vi "C_CAN_Serialize.vi"(6 "brs":bool, 7 "ide":bool, 8 "error in (no error)":errorcluster, 9 "fdf":bool, 10 "id":u32 format="%.0x", 11 "data":u8[](array[numeric]) format="%.0x") -> (0 "error out":errorcluster, 3 "payload":u8[](array[numeric]) format="%.0x")   [LabVIEW 2021, in "CANsub_C.lvlib"]
doc: "Serializes one CAN or CAN FD frame into the CANsub transmit payload (header + data). Classic: at most 8 data bytes. FD: at most 64, zero-padded to the next FD length. Standard IDs are masked to 11 bits."
uses:
  CANsub_C.lvlib
  codec_vis/CANsub_Codec.lvlib
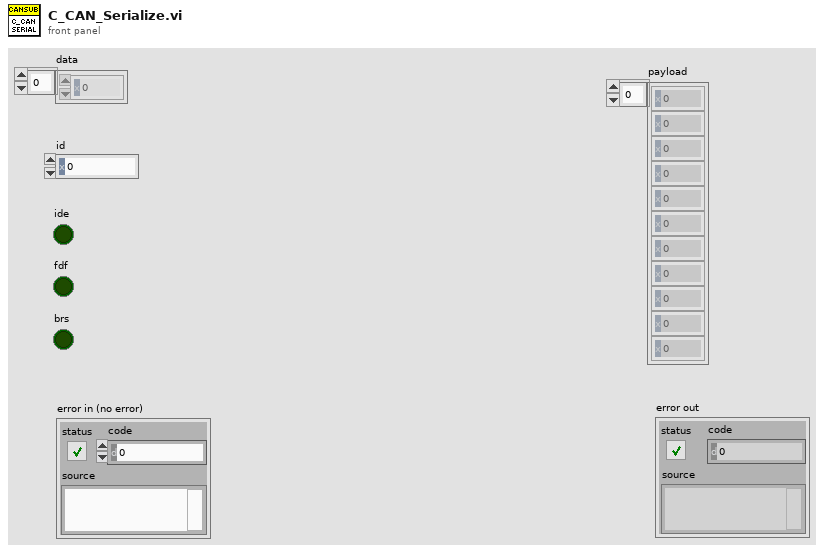
[diagram p1: front panel]
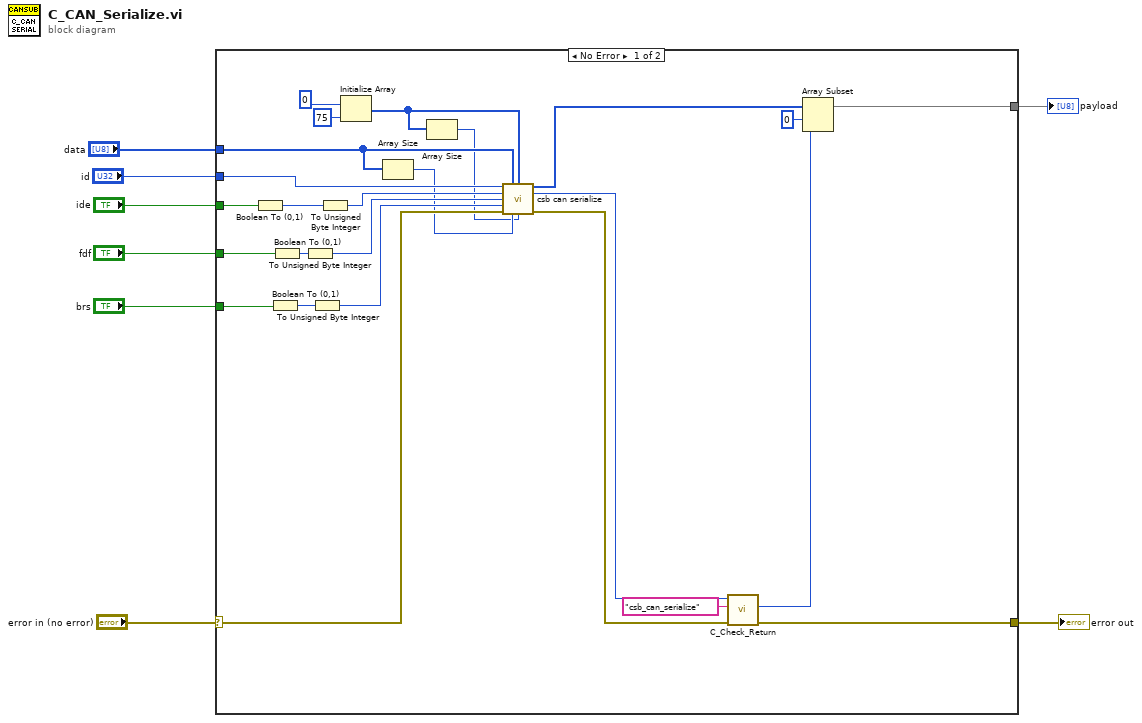
[diagram p0: block diagram]
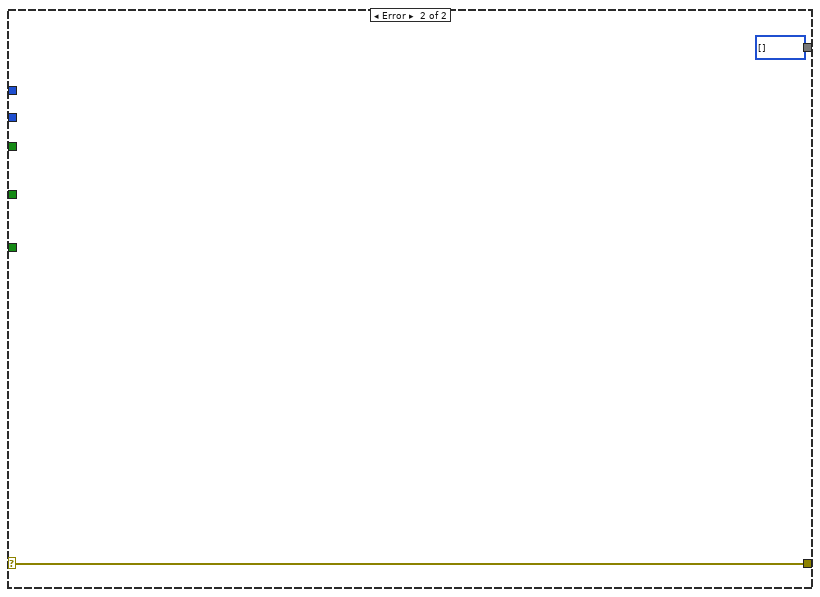
[diagram p2: hidden frame]
diagram:
  n1 = case shown="No Error" "error in (no error)" {
    selector: "error in (no error)" -> [w31 w35]
    tunnel: [w29 w35] -> w7
    tunnel: [w11 u8[] [] ("payload")] -> w6
    tunnel: "ide" -> [w26 _]
    tunnel: "fdf" -> [w25 _]
    tunnel: "brs" -> [w24 _]
    tunnel: "id" -> [w17 _]
    tunnel: "data" -> [w15 _]
    frame No Error {
      n2 = Boolean To (0,1)(Boolean=w26) -> (0, 1=w21:i16)
      n3 = Boolean To (0,1)(Boolean=w24) -> (0, 1=w23:i16)
      n4 = Boolean To (0,1)(Boolean=w25) -> (0, 1=w22:i16)
      n5 = To Unsigned Byte Integer(number=w22) -> (unsigned 8bit integer=w18:u8)
      n6 = To Unsigned Byte Integer(number=w23) -> (unsigned 8bit integer=w19:u8)
      n7 = To Unsigned Byte Integer(number=w21) -> (unsigned 8bit integer=w20:u8)
      n8 = Initialize Array(u8 0, 75 ("dimension size")) -> (w13:u8[])
      n9 = Array Size(array=w15) -> (size(s)=w14:i32)
      n10 = Array Size(array=w13) -> (size(s)=w12:i32)
      n11 = call "csb can serialize.vi"("id"=w17, "data"=w15, "payload"=w13, "ide"=w20, "fdf"=w18, "brs"=w19, "error in (no error)"=w31, "len"=w14, "payload_cap"=w12) -> ("payload out"=w16:u8[], "function return"=w28:i32, "error out"=w30:errorcluster)  [unwired: 4 in]
      n12 = call "C_Check_Return.vi"("error in (no error)"=w30, "function name"="csb_can_serialize", "function return"=w28) -> ("error out"=w29:errorcluster, "length"=w9:i32)  [unwired: 6 in, 1 out]
      n13 = Array Subset(array=w16, index=0, length=w9) -> (w11:u8[])
    }
    frame Error {
    }
  }
  "error out" <- w7
  "payload" <- w6
